vi "Generate_Rows.vi"(0 "Orientation":enum16{"Run Along Length", "Run Along Width"}(ring), 4 "Row Spacing":dbl=3.0, 5 "Field Length":dbl=8.0, 6 "Field Width":dbl=10.0) -> (1 "Waypoints":cluster{"X":dbl, "Y":dbl, "Seed":bool}[][](array[cluster]))   [LabVIEW 2022]
doc: "Rows start at origin; Width=X, Length=Y; bounded row count; incoming segment seed flags."
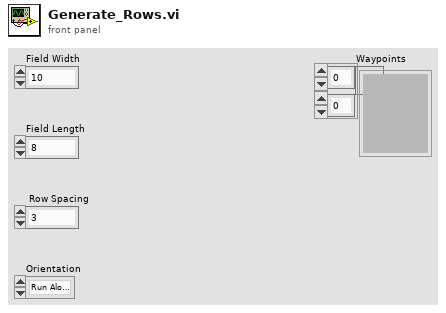
[diagram p1: front panel]
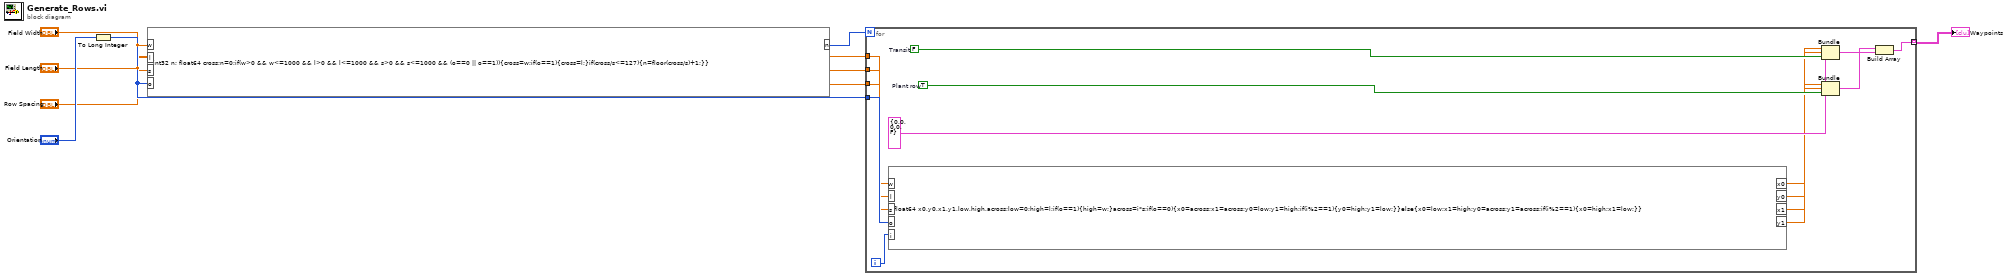
[diagram p0: block diagram]
diagram:
  n1 = To Long Integer(number="Orientation") -> (32bit integer=w5:i32[])
  n2 = formula code="int32 n; float64 cross;n=0;if(w>0 && w<=1000 && l>0 && l<=1000 && s>0 && s<=1000 && (o==0 || o==1)){cross=w;if(o==1){cross=l;}if(cross/s<=127){n=floor(cross/s)+1;}}"("w"="Field Width", "l"="Field Length", "s"="Row Spacing", "o"=w5) -> ("n"=w6:i32)
  n3 = for {
    N: w6 -> [_]
    tunnel: "Field Width" -> [w9]
    tunnel: "Field Length" -> [w10]
    tunnel: "Row Spacing" -> [w11]
    tunnel: w5 -> [w12]
    tunnel: [w22] -> w7 mode=indexing
    i -> [w8]
    w19 = cluster{"X":dbl, "Y":dbl, "Seed":bool} {"X"=0.0, "Y"=0.0, "Seed"=FALSE}
    w18 = TRUE  # Plant row
    w17 = FALSE  # Transit
    n4 = formula code="float64 x0,y0,x1,y1,low,high,across;low=0;high=l;if(o==1){high=w;}across=i*s;if(o==0){x0=across;x1=across;y0=low;y1=high;if(i%2==1){y0=high;y1=low;}}else{x0=low;x1=high;y0=across;y1=across;if(i%2==1){x0=high;x1=low;}}"("w"=w9, "l"=w10, "s"=w11, "o"=w12, "i"=w8) -> ("x0"=w13:dbl, "y0"=w14:dbl, "x1"=w15:dbl, "y1"=w16:dbl)
    n5 = Bundle(cluster=w19, "X"=w13, "Y"=w14, "Seed"=w17) -> (w20:cluster{"X":dbl, "Y":dbl, "Seed":bool})
    n6 = Bundle(cluster=w19, "X"=w15, "Y"=w16, "Seed"=w18) -> (w21:cluster{"X":dbl, "Y":dbl, "Seed":bool})
    n7 = Build Array(w20, w21) -> (w22:cluster{"X":dbl, "Y":dbl, "Seed":bool}[])
  }
  "Waypoints" <- w7
